vi "Check_Open.vi"(8 "error in (no error)":errorcluster, 11 "status":T1) -> (0 "error out":errorcluster)   [LabVIEW 2021, in "CANsub_API.lvlib"]
doc: "API private: error 5202 if the channel is Closed, 5203 if Lost; passes the error through when Open. Loop-safe: no allocation, bounded time."
uses:
  CANsub_API.lvlib
  Typedefs/CANsub_State.ctl
  common/Typedefs/Bit_Timing.ctl
  common/CANsub_Common.lvlib
  Typedefs/CANsub_Status.ctl
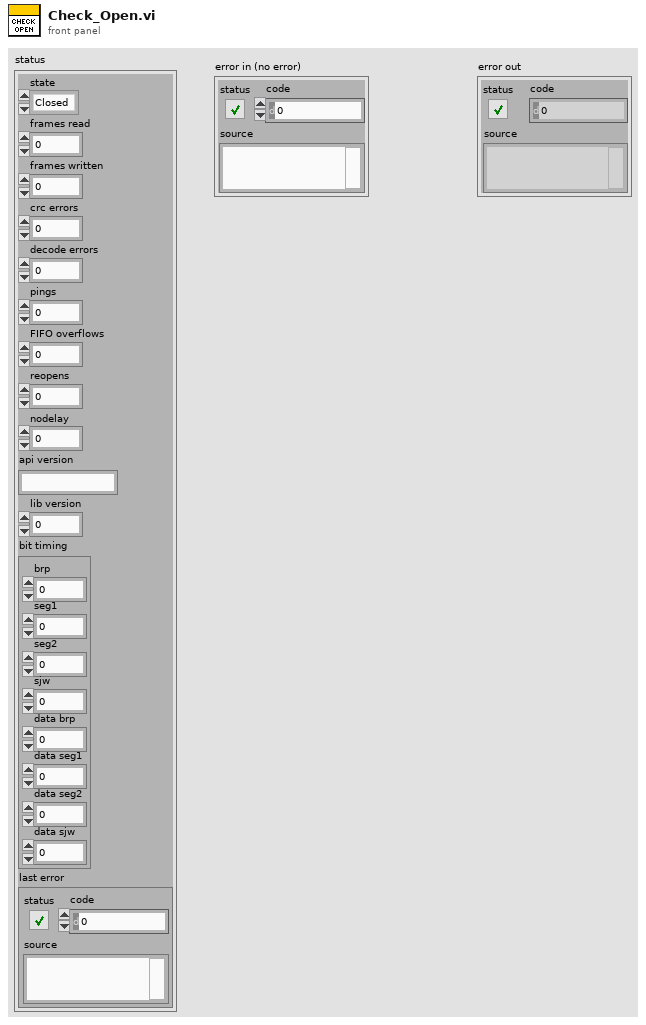
[diagram p1: front panel]
types:
  T1 = typedef "CANsub_API.lvlib/CANsub_Status.ctl" = cluster{"state":T2, "frames read":u32, "frames written":u32, "crc errors":u32, "decode errors":i32, "pings":u32, "FIFO overflows":u32, "reopens":u32, "nodelay":i32, "api version":string, "lib version":u32, "bit timing":T3, "last error":errorcluster}
  T2 = typedef "CANsub_API.lvlib/CANsub_State.ctl" = enum16{"Closed", "Open", "Lost"}
  T3 = typedef "CANsub_Common.lvlib/Bit_Timing.ctl" = cluster{"brp":u16, "seg1":u16, "seg2":u16, "sjw":u16, "data brp":u16, "data seg1":u16, "data seg2":u16, "data sjw":u16}
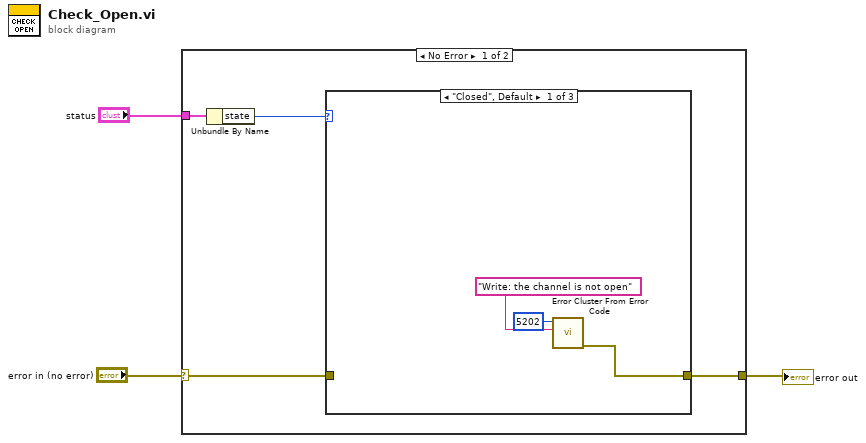
[diagram p0: block diagram]
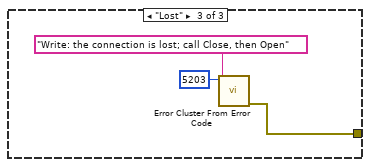
[diagram p3: hidden frame]
diagram:
  n1 = case shown="No Error" "error in (no error)" {
    selector: "error in (no error)" -> [w4 w15]
    tunnel: [w5 w15] -> w2
    tunnel: "status" -> [w7 _]
    frame No Error {
      n2 = Unbundle By Name(w7) -> ("state"=w6:T2)
      n3 = case shown="\"Closed\", Default" w6 {
        tunnel: [w9 w11 w14] -> w5
        tunnel: w4 -> [_ w11 _]
        frame "Closed", Default {
          n4 = call <vilib>:"Error Cluster From Error Code.vi"("error message (\"\")"="Write: the channel is not open" ("error message (\"\")"), "error code (0)"=5202) -> ("error out"=w9:errorcluster)  [unwired: 7 in]
        }
        frame "Open" {
        }
        frame "Lost" {
          n5 = call <vilib>:"Error Cluster From Error Code.vi"("error message (\"\")"="Write: the connection is lost; call Close, then Open" ("error message (\"\")"), "error code (0)"=5203) -> ("error out"=w14:errorcluster)  [unwired: 7 in]
        }
      }
    }
    frame Error {
    }
  }
  "error out" <- w2
